vi "Find MinMax.vi"(8 "MIN":dbl, 9 "MAX":dbl, 10 "Scale_Y":dbl, 11 "Supply Pressure":u32) -> (2 "Min output":dbl, 3 "Max output":dbl)   [LabVIEW 2025, in "Flow Grind.lvlib" / "No Load Drift.lvclass"]
uses:
  No Load Drift.lvclass
  No Load Drift.lvclass/No Load Drift.ctl
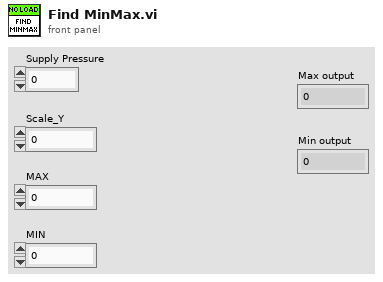
[diagram p1: front panel]
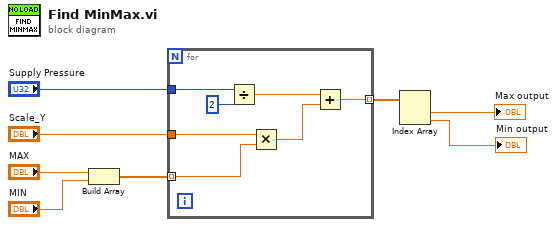
[diagram p0: block diagram]
diagram:
  n1 = Build Array("MAX", "MIN") -> (w5:dbl[])
  n2 = for {
    tunnel: "Supply Pressure" -> [w12]
    tunnel: "Scale_Y" -> [w11]
    tunnel: w5 -> [w10] mode=indexing
    tunnel: [w9] -> w3 mode=indexing
    n3 = Divide(x=w12, y=u32 2) -> (x/y=w14:dbl)
    n4 = Multiply(x=w11, y=w10) -> (x*y=w13:dbl)
    n5 = Add(x=w14, y=w13) -> (x+y=w9:dbl)
  }
  n6 = Index Array(array=w3) -> (element #1=→"Max output":dbl, element #2=→"Min output":dbl)  [unwired: 2 in]
